vi "GetTestTypeDescv2NoRbac.vi"() -> ()   [LabVIEW 2017]
uses:
  <vilib>/httpClient/POSTBuffer.vi
  <vilib>/httpClient/LabVIEWHTTPClient.lvlib
  <vilib>/Analysis/NI_AALBase.lvlib
panel:
  out "standard deviation":dbl format="%0.2f"
  out "mean":dbl format="%0.2f"
  out "error out":errorcluster
  out "test_property":T1
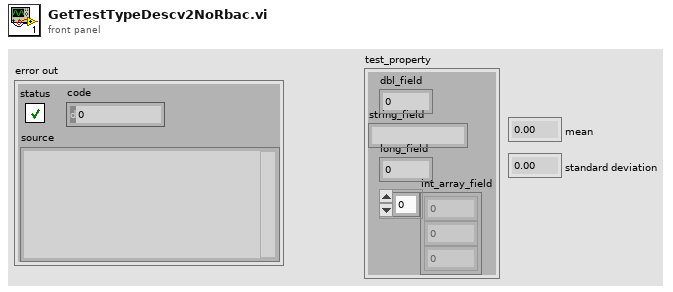
[diagram p1: front panel]
types:
  T1 = cluster{"dbl_field":dbl, "string_field":string, "long_field":i64, "int_array_field":i32[]}
  T2 = cluster{"req_action":string, "selector":string, "req_lang":string, "device":string, "type_descriptor":i16[]}
  T3 = typedef "LabVIEWHTTPClient.lvlib/ClientHandle.ctl" = refnum<k1>
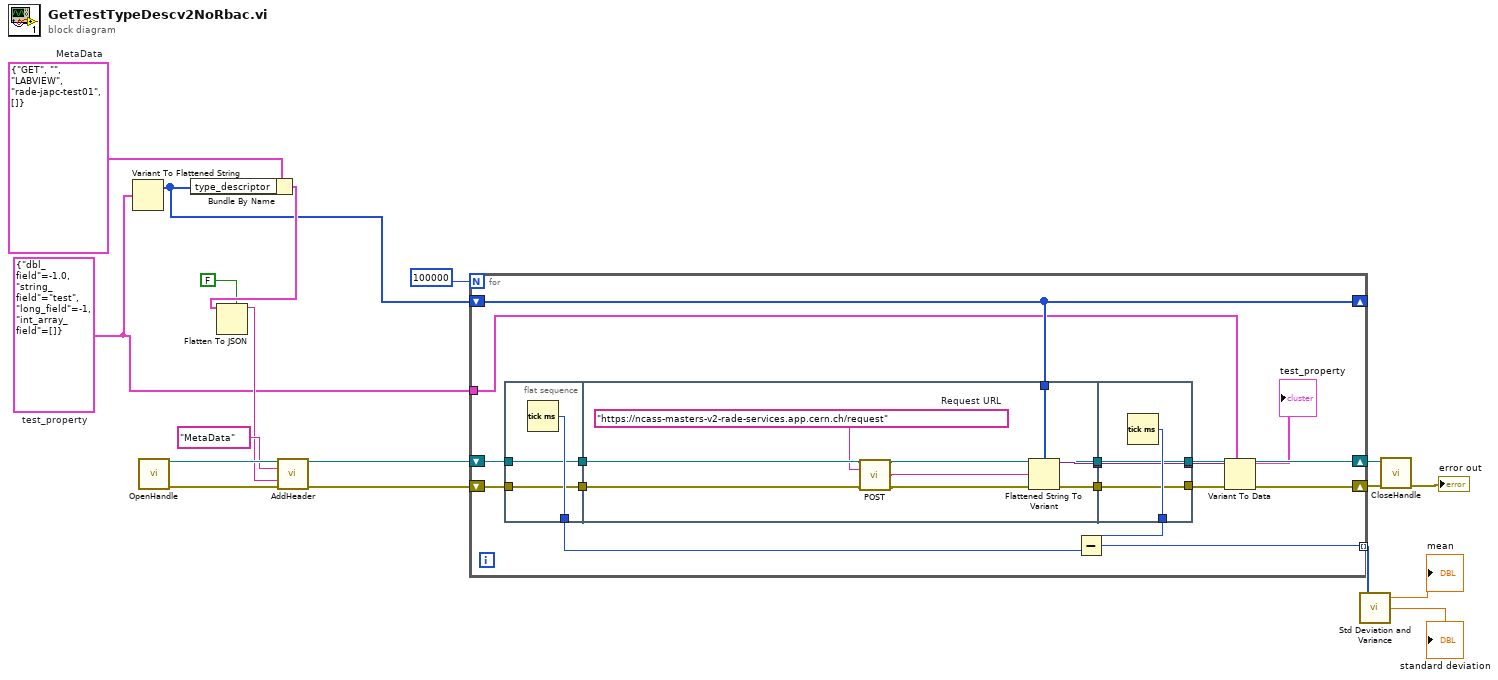
[diagram p0: block diagram]
diagram:
  w6 = T2 {"req_action"="GET", "selector"="", "req_lang"="LABVIEW", "device"="rade-japc-test01", "type_descriptor"=[]}  # MetaData
  w2 = T1 {"dbl_field"=-1.0, "string_field"="test", "long_field"=-1, "int_array_field"=[]}  # test_property
  n1 = Variant To Flattened String(Variant=w2) -> (1:w1:i16[])  [unwired: 1 out]
  n2 = call <vilib>:"OpenHandle.vi"() -> ("client handle out"=w16:T3, "error out"=w17:errorcluster)  [unwired: 14 in]
  n3 = Bundle By Name(cluster=w6, "type_descriptor"=w1) -> (w5:T2)
  n4 = Flatten To JSON(enable LabVIEW extensions? (T)=FALSE, anything=w5) -> (JSON string=w3:string)  [unwired: 1 in, 1 out]
  n5 = call <vilib>:"AddHeader.vi"("client handle"=w16, "header"="MetaData", "value"=w3, "error in (no error)"=w17) -> ("client handle out"=w8:T3, "error out"=w7:errorcluster)  [unwired: 10 in]
  n6 = for {
    N: 100000 -> [_]
    shift-right: [w35] -> _
    shift-left: w1 -> [w35]
    tunnel: w2 -> [w30]
    tunnel: [w26] -> w11 mode=indexing
    shift-right: [w28] -> w13
    shift-left: w8 -> [w24]
    shift-right: [w19] -> w12
    shift-left: w7 -> [w22]
    n7 = flat-sequence {
      tunnel: [w38] -> w34
      tunnel: [w37] -> w25
      tunnel: w24 -> [w37]
      tunnel: [w36] -> w23
      tunnel: w22 -> [w36]
      tunnel: w35 -> [w47]
      tunnel: [w46] -> w32
      tunnel: [w40] -> w29
      tunnel: [w45] -> w27
      tunnel: w25 -> [w44]
      tunnel: w23 -> [w43]
      tunnel: [w51] -> w33
      tunnel: w32 -> [w50]
      tunnel: [w50] -> w31
      tunnel: [w49] -> w28
      tunnel: w29 -> [w49]
      tunnel: [w48] -> w20
      tunnel: w27 -> [w48]
      frame #0 {
        n8 = Tick Count (ms)() -> (millisecond timer value=w38:u32)
      }
      frame #1 {
        w39 = "https://ncass-masters-v2-rade-services.app.cern.ch/request"  # Request URL
        n9 = call-poly <vilib>:"POST.vi"("client handle"=w44, "url"=w39, "error in (no error)"=w43) -> ("client handle out"=w40:T3, "body"=w41:string, "error out"=w42:errorcluster)  [unwired: 9 in, 1 out]
        n10 = Flattened String To Variant(4:w42, 6:w41, 7:w47) -> (0:w45:errorcluster, 3:w46:variant)
      }
      frame #2 {
        n11 = Tick Count (ms)() -> (millisecond timer value=w51:u32)
      }
    }
    n12 = Subtract(x=w33, y=w34) -> (x-y=w26:u32)
    n13 = Variant To Data(error in=w20, type=w30, Variant=w31) -> (data=→"test_property":T1, error out=w19:errorcluster)
  }
  n14 = call <vilib>:"Std Deviation and Variance.vi"("X"=w11) -> ("mean"=→"mean":dbl, "standard deviation"=→"standard deviation":dbl)  [unwired: 1 in, 1 out]
  n15 = call <vilib>:"CloseHandle.vi"("client handle"=w13, "error in (no error)"=w12) -> ("error out"=→"error out":errorcluster)  [unwired: 13 in]
